vi "Read XML Document.vi"(8 "error in (no error)":errorcluster, 11 "ToastFromXML in":refnum<class "ToastFromXML.lvclass">) -> (0 "error out":errorcluster, 2 "XML Document":refnum<k24>, 3 "ToastFromXML out":refnum<class "ToastFromXML.lvclass">)   [LabVIEW 2026, in "ToastNotification.lvlib" / "ToastFromXML.lvclass"]
doc: "Read the private XML Document reference through the class property. Returns a borrowed alias; no new ownership is acquired. Skipped on incoming error. Internal accessor; use Get XML for application XML export."
uses:
  ToastFromXML.lvclass
  ToastFromXML.lvclass/ToastFromXML.ctl
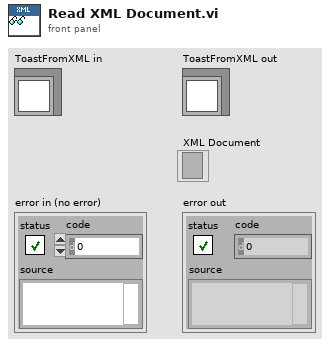
[diagram p1: front panel]
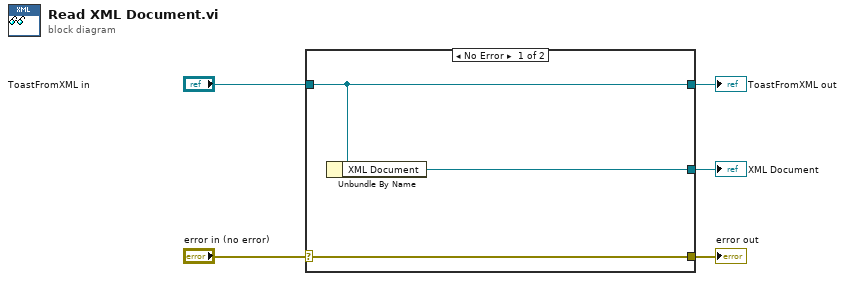
[diagram p0: block diagram]
diagram:
  n1 = case shown="No Error" "error in (no error)" {
    selector: "error in (no error)" -> [w8 w9]
    tunnel: [w8 w9] -> w4
    tunnel: [w7 w10] -> w2
    tunnel: "ToastFromXML in" -> [w7 w10]
    tunnel: [w6 _] -> w1
    frame No Error {
      n2 = Unbundle By Name(w7) -> ("XML Document"=w6:refnum<k24>)
    }
    frame Error {
    }
  }
  "error out" <- w4
  "ToastFromXML out" <- w2
  "XML Document" <- w1
